vi "Enable_Motor.vi"(8 "error in (no error)":errorcluster, 10 "Enable Drive":bool=TRUE, 11 "Motor in":refnum<class "Motor.lvclass">) -> (0 "error out":errorcluster, 3 "Motor out":refnum<class "Motor.lvclass">)   [LabVIEW 2021, in "Motor.lvclass"]
uses:
  Motor.lvclass
  Motor.lvclass/Motor.ctl
  ServoDrive/ServoDrive.lvclass
  AnalogOutput/AnalogOutput.lvclass
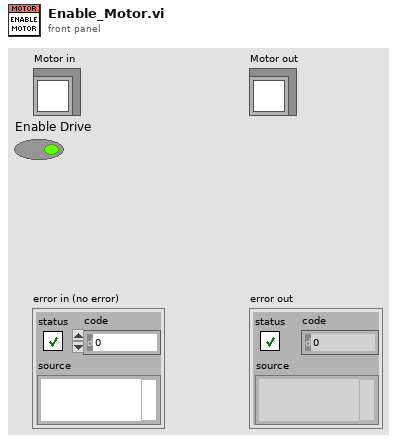
[diagram p1: front panel]
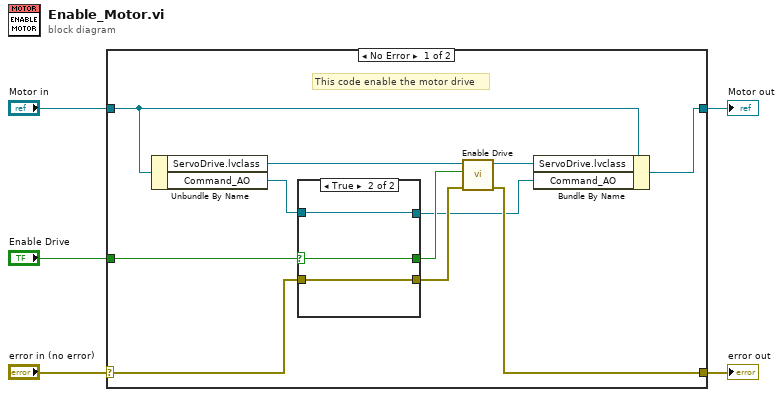
[diagram p0: block diagram]
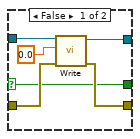
[diagram p2: hidden frame]
diagram:
  n1 = case shown="No Error" "error in (no error)" {
    selector: "error in (no error)" -> [w10 w27]
    tunnel: [w12 w27] -> w4
    tunnel: [w14 w26] -> w2
    tunnel: "Motor in" -> [w15 w26]
    tunnel: "Enable Drive" -> [w8 _]
    frame No Error {
      # "This code enable the motor drive"
      n2 = Unbundle By Name(w15) -> ("ServoDrive.lvclass"=w16:refnum<class "ServoDrive.lvclass">, "Command_AO"=w11:refnum<class "AnalogOutput.lvclass">)
      n3 = case shown="True" w8 {
        selector: w8 -> [w18 w24]
        tunnel: w11 -> [w21 w23]
        tunnel: w10 -> [w20 w25]
        tunnel: [w19 w25] -> w9
        tunnel: [w18 w24] -> w7
        tunnel: [w17 w23] -> w6
        frame False {
          n4 = call-dynamic "Write.vi"("error in (no error)"=w20, "data in"=0.0, "AnalogOutput in"=w21) -> ("error out"=w19:errorcluster, "AnalogOutput out"=w17:refnum<class "AnalogOutput.lvclass">)  [unwired: 7 in]
        }
        frame True {
        }
      }
      n5 = call-dynamic "Enable Drive.vi"("error in (no error)"=w9, "Enable Drive"=w7, "ServoDrive in"=w16) -> ("error out"=w12:errorcluster, "ServoDrive out"=w13:refnum<class "ServoDrive.lvclass">)  [unwired: 7 in]
      n6 = Bundle By Name(cluster=w15, "ServoDrive.lvclass"=w13, "Command_AO"=w6) -> (w14:refnum<class "Motor.lvclass">)
    }
    frame Error {
    }
  }
  "error out" <- w4
  "Motor out" <- w2
